vi "Main.vi"() -> ()   [LabVIEW 2018]
uses:
  <vilib>/vision/Image Controls.llb/IMAQ Image.ctl
  <vilib>/vision/NI_Vision_Development_Module.lvlib
panel:
  out "мВ":dbl
  out "DSNU, мВ":dbl
  out "WHITE_COLUMN":i32
  out "Waveform Graph":T1(graph)={"Starting Value"=0.0, "Incremental Value"=131.072, [0.0, 0.0, 0.0, 0.0, 0.0, 0.00020469500207774904, 0.012080795770773818, 0.30584607978272005, 0.418065850192636, 0.25104752193482266, 0.013277219104677327, 0.00043639837248520105, 0.0004392413586251698, 5.8281215869359104e-05, 1.4214930699843683e-06, 9.476620466562456e-07, 4.738310233281228e-07, 0.0, 0.0, 0.0, 0.0, 0.0, 0.0, 0.0, 0.0, 0.0, 0.0, 0.0, 0.0, 0.0, 0.0, 0.0, 0.0, 0.0, 0.0, 0.0, 0.0, 0.0, 0.0, 0.0, 0.0, 0.0, 0.0, 0.0, 0.0, 0.0, 0.0, 0.0, 0.0, 0.0, 0.0, 0.0, 0.0, 0.0, 0.0, 0.0, 0.0, 0.0, 0.0, 0.0, 0.0, 0.0, 0.0, 0.0, 0.0, 0.0, 0.0, 0.0, 0.0, 0.0, 0.0, 0.0, 0.0, 0.0, 0.0, 0.0, 0.0, 0.0, 0.0, 0.0, 0.0, 0.0, 0.0, 0.0, 0.0, 0.0, 0.0, 0.0, 0.0, 0.0, 0.0, 0.0, 0.0, 0.0, 0.0, 0.0, 0.0, 0.0, 0.0, 0.0, 0.0, 0.0, 0.0, 0.0, 0.0, 0.0, 0.0, 0.0, 0.0, 0.0, 0.0, 0.0, 0.0, 0.0, 0.0, 0.0, 0.0, 0.0, 0.0, 0.0, 0.0, 0.0, 0.0, 0.0, 0.0, 0.0, 0.0, 0.0, 0.0, 0.0, 0.0, 0.0, 0.0, 0.0, 0.0, 0.0, 0.0, 0.0, 0.0, 0.0, 0.0, 0.0, 0.0, 0.0, 0.0, 0.0, 0.0, 0.0, 0.0, 0.0, 0.0, 0.0, 0.0, 0.0, 0.0, 0.0, 0.0, 0.0, 0.0, 0.0, 0.0, 0.0, 0.0, 0.0, 0.0, 0.0, 0.0, 0.0, 0.0, 0.0, 0.0, 0.0, 0.0, 0.0, 0.0, 0.0, 0.0, 0.0, 0.0, 0.0, 0.0, 0.0, 0.0, 0.0, 0.0, 0.0, 0.0, 0.0, 0.0, 0.0, 0.0, 0.0, 0.0, 0.0, 0.0, 0.0, 0.0, 0.0, 0.0, 0.0, 0.0, 0.0, 0.0, 0.0, 0.0, 0.0, 0.0, 0.0, 0.0, 0.0, 0.0, 0.0, 0.0, 0.0, 0.0, 0.0, 0.0, 0.0, 0.0, 0.0, 0.0, 0.0, 0.0, 0.0, 0.0, 0.0, 0.0, 0.0, 0.0, 0.0, 0.0, 0.0, 0.0, 0.0, 0.0, 0.0, 0.0, 0.0, 0.0, 0.0, 0.0, 0.0, 0.0, 0.0, 0.0, 0.0, 0.0, 0.0, 0.0, 0.0, 0.0, 0.0, 0.0, 0.0, 0.0, 0.0, 0.0, 0.0, 0.0, 0.0, 0.0, 0.0, 0.0, 0.0, 0.0, 0.0, 0.0, 0.0, 0.0, 0.0, 0.0, 0.0, 0.0, 0.0, 0.0, 0.0, 0.0, 0.0, 0.0, 0.0, 0.0, 0.0, 0.0, 0.0, 0.0, 0.0, 0.0, 0.0, 0.0, 0.0, 0.0, 0.0, 0.0, 0.0, 0.0, 0.0, 0.0, 0.0, 0.0, 0.0, 0.0, 0.0, 0.0, 0.0, 0.0, 0.0, 0.0, 0.0, 0.0, 0.0, 0.0, 0.0, 0.0, 0.0, 0.0, 0.0, 0.0, 0.0, 0.0, 0.0, 0.0, 0.0, 0.0, 0.0, 0.0, 0.0, 0.0, 0.0, 0.0, 0.0, 0.0, 0.0, 0.0, 0.0, 0.0, 0.0, 0.0, 0.0, 0.0, 0.0, 0.0, 0.0, 0.0, 0.0, 0.0, 0.0, 0.0, 0.0, 0.0, 0.0, 0.0, 0.0, 0.0, 0.0, 0.0, 0.0, 0.0, 0.0, 0.0, 0.0, 0.0, 0.0, 0.0, 0.0, 0.0, 0.0, 0.0, 0.0, 0.0, 0.0, 0.0, 0.0, 0.0, 0.0, 0.0, 0.0, 0.0, 0.0, 0.0, 0.0, 0.0, 0.0, 0.0, 0.0, 0.0, 0.0, 0.0, 0.0, 0.0, 0.0, 0.0, 0.0, 0.0, 0.0, 0.0, 0.0, 0.0, 0.0, 0.0, 0.0, 0.0, 0.0, 0.0, 0.0, 0.0, 0.0, 0.0, 0.0, 0.0, 0.0, 0.0, 0.0, 0.0, 0.0, 0.0, 0.0, 0.0, 0.0, 0.0, 0.0, 0.0, 0.0, 0.0, 0.0, 0.0, 0.0, 0.0, 0.0, 0.0, 0.0, 0.0, 0.0, 0.0, 0.0, 0.0, 0.0, 0.0, 0.0, 0.0, 0.0, 0.0, 0.0, 0.0, 0.0, 0.0, 0.0, 0.0, 0.0, 0.0, 0.0, 0.0, 0.0, 0.0, 0.0, 0.0, 0.0, 0.0, 0.0, 0.0, 0.0, 0.0, 0.0, 0.0, 0.0, 0.0, 0.0, 0.0, 0.0, 0.0, 0.0, 0.0, 0.0, 0.0, 0.0, 0.0, 0.0, 0.0, 0.0, 0.0, 0.0, 0.0, 0.0, 0.0, 0.0, 0.0, 0.0, 0.0, 0.0, 0.0, 0.0, 0.0, 0.0, 0.0, 0.0, 0.0, 0.0, 0.0, 0.0, 0.0, 0.0]}
  in  "Interval Range":cluster{"Minimum":sgl, "Maximum":sgl}={"Minimum"=0.0, "Maximum"=5000.0} {"Maximum" format="%.2f"; "Minimum" format="%.2f"}
  in  "Image Mask":T2
  in  "Number of Classes":i32=500
  out "ЧБД":i32
  out "БД":i32
  out "ЧД":i32
  in  "Uнас, мВ":dbl=1500.0 format="%#_13g"
  out "Среднее \nвсего \nкадра":dbl=1101.1682678206664
  out "Кол-во пикселей":i32=2110457
  out "Среднее\nвыделенной":dbl=nan
  out "Image":T2(plugin-control)
  in  "File Path":path=path "C:/VPL/LabView_PRJ/ФППЗ_1024М/FRAMES/17/Темно/СТАРЫЕ/ДЕФЕКТЫ/ТЕМ1_Тн5_Nk5_рад_10.54.30.tiff"
  in  "Старт":bool
  in  "Стоп":bool
  out "x+y":dbl
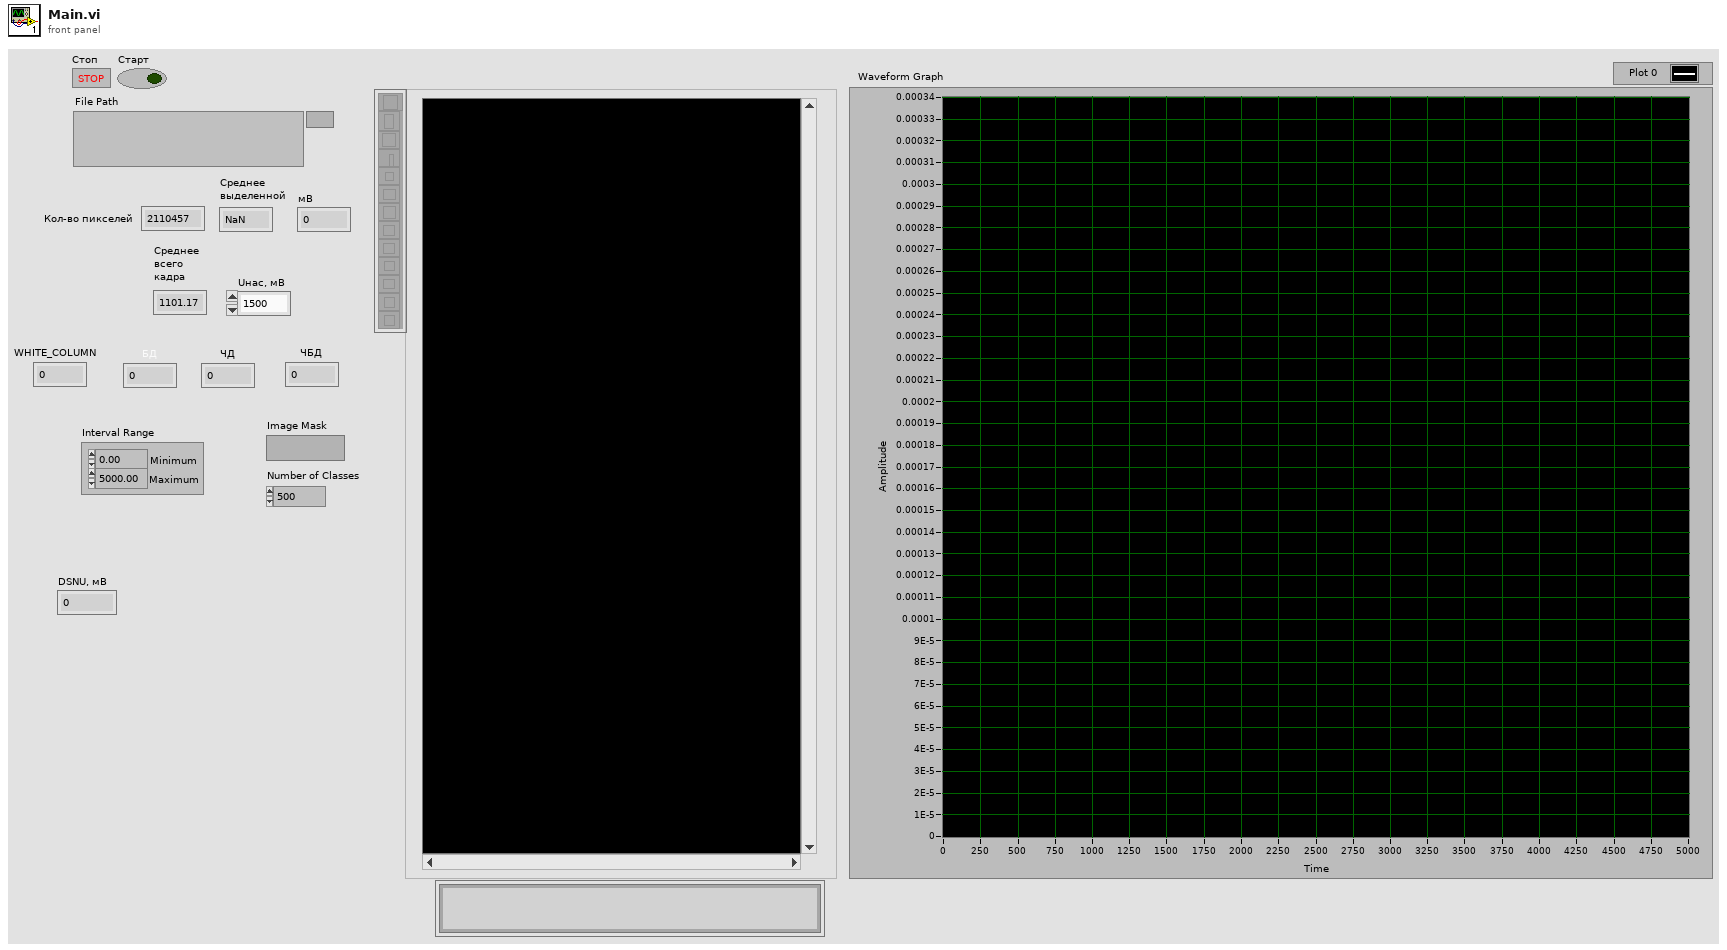
[diagram p1: front panel]
types:
  T1 = cluster{"Starting Value":sgl, "Incremental Value":sgl, dbl[]}
  T2 = typedef "IMAQ Image.ctl" = refnum<image>
  T3 = typedef "Image Type" = u32
  T4 = cluster{"Global Rectangle":i32[], "Contours":cluster{"Contour Type":u32, "ROI Type":u32, "Points":i32[]}[]}
  T5 = cluster{"Contour Type":u32, "ROI Type":u32, "Points":i32[]}[]
  T6 = cluster{"Contour Type":u32, "ROI Type":u32, "Points":i32[]}
  T7 = cluster{"Starting Value":sgl, "Incremental Value":sgl, "Histogram":u32[]}
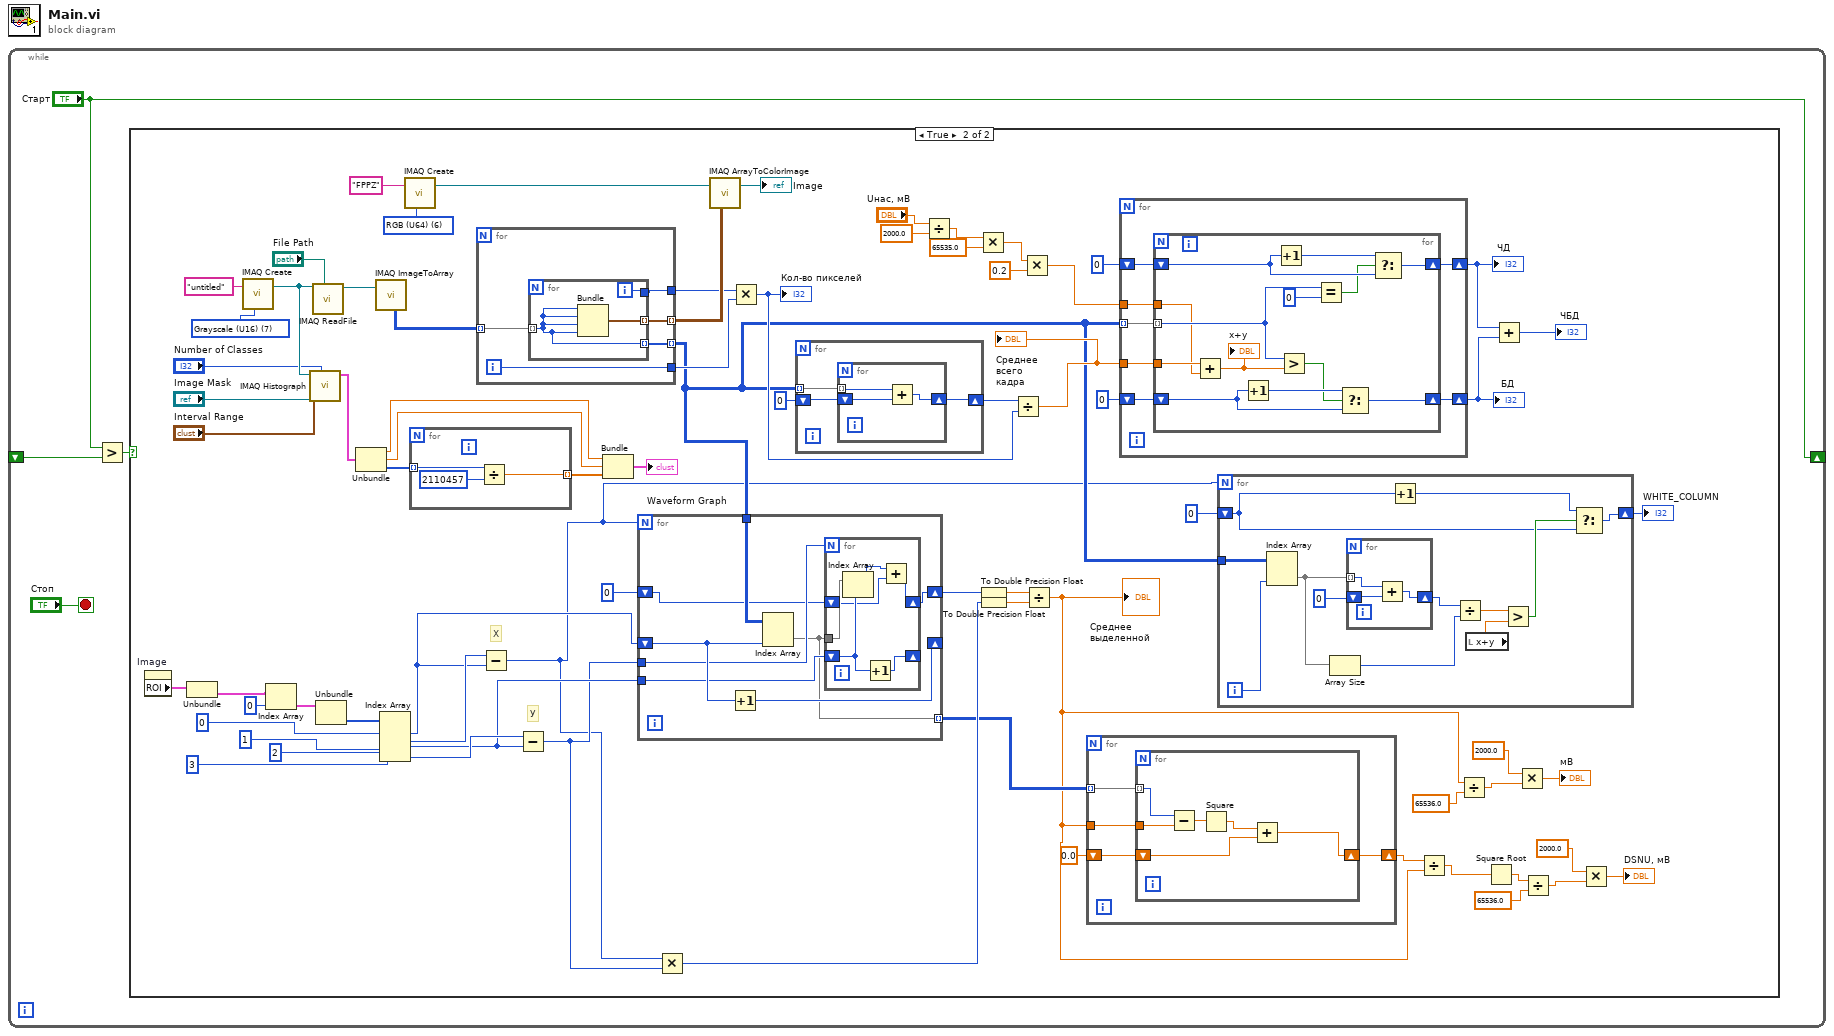
[diagram p0: block diagram]
diagram:
  n1 = while {
    shift-right: ["Старт"] -> _
    shift-left: _ -> [w3]
    stop <- "Стоп" stop-if-true
    n2 = Greater?(x="Старт", y=w3) -> (0:w1:bool)
    n3 = case shown="True" w1 {
      frame False {
      }
      frame True {
        w75 = T3 6 items=["Grayscale (U8)", "Grayscale (I16)", "Grayscale (SGL)", "Complex (CSG)", "RGB (U32)", "HSL (U32)", "RGB (U64)"] ("Image Type")
        w78 = T3 7 items=["Grayscale (U8)", "Grayscale (I16)", "Grayscale (SGL)", "Complex (CSG)", "RGB (U32)", "HSL (U32)", "RGB (U64)", "Grayscale (U16)"] ("Image Type")
        # "У"
        # "Х"
        n4 = property on="Image" class="ImageControl"() -> ("ROI"=w72:T4)  [unwired: 2 in, 2 out]
        n5 = Unbundle(w72) -> ("Contours"=w71:T5)  [unwired: 1 out]
        n6 = call "IMAQ Create"("Image Name"="untitled", "Image Type"=w78) -> ("New Image"=w34:T2)  [unwired: 3 in, 1 out]
        n7 = Index Array(array=w71, index=0) -> (element=w69:T6)
        n8 = call "IMAQ Histograph"("Number of Classes"="Number of Classes", "Interval Range"="Interval Range", "Image Mask"="Image Mask", "Image"=w34) -> ("Histogram Graph"=w30:T7)  [unwired: 4 in, 3 out]
        n9 = call "IMAQ ReadFile"("File Path"="File Path", "Image"=w34) -> ("Image Out"=w35:T2)  [unwired: 5 in, 4 out]
        n10 = Unbundle(w69) -> ("Points"=w68:i32[])  [unwired: 2 out]
        n11 = Unbundle(w30) -> ("Starting Value"=w28:sgl, "Incremental Value"=w27:sgl, "Histogram"=w29:u32[])
        n12 = call "IMAQ ImageToArray"("Image"=w35) -> ("Image Pixels (U16)"=w77:u16[][])  [unwired: 3 in, 4 out]
        n13 = Index Array(array=w68, index #1=0 ("index"), index #2=2 ("index"), index #3=1 ("index"), index #4=3 ("index")) -> (element #1=w60:i32, element #2=w61:i32, element #3=w59:i32, element #4=w62:i32)
        n14 = call "IMAQ Create"("Image Name"="FPPZ", "Image Type"=w75) -> ("New Image"=w74:T2)  [unwired: 3 in, 1 out]
        n15 = for {
          tunnel: w29 -> [w107] mode=indexing
          tunnel: [w105] -> w26 mode=indexing
          n16 = Divide(x=w107, y=u32 2110457) -> (x/y=w105:dbl)
        }
        n17 = for {
          tunnel: w77 -> [w152] mode=indexing
          tunnel: [w151] -> w76 mode=indexing
          tunnel: [w150] -> w22 mode=indexing
          tunnel: [w149] -> w53
          tunnel: [w148] -> w52
          i -> [w148]
          n18 = for {
            tunnel: w152 -> [w154] mode=indexing
            tunnel: [w155] -> w151 mode=indexing
            tunnel: [w154] -> w150 mode=indexing
            tunnel: [w153] -> w149
            i -> [w153]
            n19 = Bundle(w154, w154, w154, w154) -> (w155:cluster{u16, u16, u16, u16})  [unwired: 1 in]
          }
        }
        n20 = Subtract(x=w61, y=w60) -> (x-y=w19:i32)
        n21 = Subtract(x=w62, y=w59) -> (x-y=w58:i32)
        n22 = Bundle("Starting Value"=w28, "Incremental Value"=w27, w26) -> (→"Waveform Graph":T1)  [unwired: 1 in]
        n23 = for {
          N: w19 -> [_]
          tunnel: w58 -> [w138]
          tunnel: w22 -> [w141]
          shift-right: [w140] -> _
          shift-left: w60 -> [w139]
          tunnel: w59 -> [w137]
          shift-right: [w135] -> w57
          shift-left: u64 0 -> [w136]
          tunnel: [w134] -> w18 mode=indexing
          n24 = Increment(x=w139) -> (x+1=w140:i32)
          n25 = Index Array(array=w141, index (col)=w139) -> (element=w134:u16[])  [unwired: 1 in]
          n26 = for {
            N: w138 -> [_]
            tunnel: w134 -> [w147]
            shift-right: [w145] -> _
            shift-left: w137 -> [w146]
            shift-right: [w142] -> w135
            shift-left: w136 -> [w143]
            n27 = Index Array(array=w147, index=w146) -> (element=w144:u16)
            n28 = Increment(x=w146) -> (x+1=w145:i32)
            n29 = Add(x=w144, y=w143) -> (x+y=w142:u64)
          }
        }
        n30 = Multiply(x=w19, y=w58) -> (x*y=w55:i32)
        n31 = call "IMAQ ArrayToColorImage"("Image"=w74, "Image Pixels (U64)"=w76) -> ("Image Out"=→"Image":T2)  [unwired: 3 in, 1 out]
        n32 = Multiply(x=w53, y=w52) -> (x*y=w50:i32)
        "Кол-во пикселей" <- w50
        n33 = for {
          tunnel: w22 -> [w130] mode=indexing
          shift-right: [w128] -> w51
          shift-left: u64 0 -> [w129]
          n34 = for {
            tunnel: w130 -> [w133] mode=indexing
            shift-right: [w131] -> w128
            shift-left: w129 -> [w132]
            n35 = Add(x=w133, y=w132) -> (x+y=w131:u64)
          }
        }
        n36 = Divide(x="Uнас, мВ", y=2000.0) -> (x/y=w45:dbl)
        n37 = Multiply(x=w45, y=65535.0) -> (x*y=w42:dbl)
        n38 = To Double Precision Float(number=w57) -> (double precision float=w56:dbl)
        n39 = To Double Precision Float(number=w55) -> (double precision float=w54:dbl)
        n40 = Divide(x=w51, y=w50) -> (x/y=w48:dbl)
        "Среднее \nвсего \nкадра" <- w48
        n41 = Multiply(x=w42, y=0.2) -> (x*y=w40:dbl)
        n42 = Divide(x=w56, y=w54) -> (x/y=w6:dbl)
        "Среднее\nвыделенной" <- w6
        n43 = for {
          tunnel: w18 -> [w83] mode=indexing
          tunnel: w6 -> [w82]
          shift-right: [w80] -> w16
          shift-left: 0.0 -> [w81]
          n44 = for {
            tunnel: w83 -> [w89] mode=indexing
            tunnel: w82 -> [w88]
            shift-right: [w84] -> w80
            shift-left: w81 -> [w85]
            n45 = Subtract(x=w89, y=w88) -> (x-y=w87:dbl)
            n46 = Square(x=w87) -> (x^2=w86:dbl)
            n47 = Add(x=w86, y=w85) -> (x+y=w84:dbl)
          }
        }
        n48 = for {
          tunnel: w22 -> [w114] mode=indexing
          tunnel: w48 -> [w113]
          tunnel: w40 -> [w111]
          shift-right: [w110] -> w38
          shift-left: 0 -> [w112]
          shift-right: [w108] -> w37
          shift-left: 0 -> [w109]
          n49 = for {
            tunnel: w114 -> [w127] mode=indexing
            tunnel: w113 -> [w126]
            tunnel: w111 -> [w125]
            shift-right: [w121] -> w110
            shift-left: w112 -> [w122]
            shift-right: [w115] -> w108
            shift-left: w109 -> [w117]
            n50 = Add(x=w126, y=w125) -> (x+y=w124:dbl)
            "x+y" <- w124
            n51 = Increment(x=w117) -> (x+1=w118:i32)
            n52 = Increment(x=w122) -> (x+1=w123:i32)
            n53 = Greater?(x=w127, y=w124) -> (0:w116:bool)
            n54 = Equal?(x=w127, y=u16 0) -> (x = y?=w119:bool)
            n55 = Select(t=w118, s=w116, f=w117) -> (s? t:f=w115:i32)
            n56 = Select(t=w123, s=w119, f=w122) -> (s? t:f=w121:i32)
          }
        }
        "ЧД" <- w38
        "БД" <- w37
        n57 = for {
          N: w19 -> [_]
          tunnel: w22 -> [w101]
          shift-right: [w90] -> w20
          shift-left: 0 -> [w91]
          i -> [w100]
          n58 = Index Array(array=w101, index (col)=w100) -> (element=w97:u16[])  [unwired: 1 in]
          n59 = Array Size(array=w97) -> (size(s)=w96:i32)
          n60 = for {
            tunnel: w97 -> [w104] mode=indexing
            shift-right: [w102] -> w98
            shift-left: 0 -> [w103]
            n61 = Add(x=w104, y=w103) -> (x+y=w102:i32)
          }
          n62 = Increment(x=w91) -> (x+1=w92:i32)
          n63 = Divide(x=w98, y=w96) -> (x/y=w95:dbl)
          n64 = local read "x+y"() -> (w94:dbl)
          n65 = Greater?(x=w95, y=w94) -> (0:w93:bool)
          n66 = Select(t=w92, s=w93, f=w91) -> (s? t:f=w90:i32)
        }
        "WHITE_COLUMN" <- w20
        n67 = Divide(x=w16, y=w6) -> (x/y=w13:dbl)
        n68 = Divide(x=w6, y=65536.0) -> (x/y=w8:dbl)
        n69 = Square Root(x=w13) -> (sqrt(x)=w15:dbl)
        n70 = Add(x=w38, y=w37) -> (x+y=→"ЧБД":i32)
        n71 = Multiply(x=2000.0, y=w8) -> (x*y=→"мВ":dbl)
        n72 = Divide(x=w15, y=65536.0) -> (x/y=w12:dbl)
        n73 = Multiply(x=2000.0, y=w12) -> (x*y=→"DSNU, мВ":dbl)
      }
    }
  }
